vi "build.iso8601.vi"(11 "seriesName":string) -> (3 "Timestamp Metadata":refnum<class "timestampMetadata.lvclass">)   [LabVIEW 2020, in "ts.iso8601.lvclass"]
uses:
  ts.iso8601.lvclass
  timestampMetadata/timestampMetadata.lvclass
  timestampMetadata/seriesName.set.vi
  timestampMetadata/timestampType.set.vi
  ts.iso8601.lvclass/ts.iso8601.ctl
  C:/code/labview-client/lv_src/ts.absoloute type/ts.absoloute type.lvclass
  C:/code/labview-client/lv_src/timestampType/timestampType.lvclass
  C:/code/labview-client/lv_src/Nominal Client/datasources/payload/payload.lvclass
  C:/code/labview-client/lv_src/ts.iso8601/ts.iso8601.lvclass
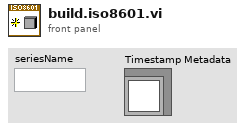
[diagram p1: front panel]
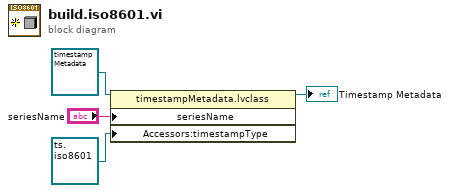
[diagram p0: block diagram]
diagram:
  n1 = property class="timestampMetadata.lvclass"(reference=refnum<class "timestampMetadata.lvclass"> refnum ("timestampMetadata.lvclass"), "seriesName"="seriesName", "Accessors:timestampType"=refnum<class "ts.iso8601.lvclass"> refnum ("ts.iso8601 in")) -> (reference out=→"Timestamp Metadata":refnum<class "timestampMetadata.lvclass">)  [unwired: 1 in, 1 out]
